vi "RemoteVI Origin Message.vi"(0 "origin":cluster{"x":i32, "y":i32}) -> (4 "frame":string)   [LabVIEW 2020, in "RemoteVI.lvlib"]
doc: "The text message origin x y (docs\\protocol.md 3.3) as a WebSocket text frame (RemoteVI WS Encode Server Frame.vi): where the panel area starts inside the frame - below the menu bar and the toolbar. Every client gets it with the greeting, and all clients again whenever it changes (RemoteVI Send Origin.vi). Pure."
uses:
  RemoteVI.lvlib
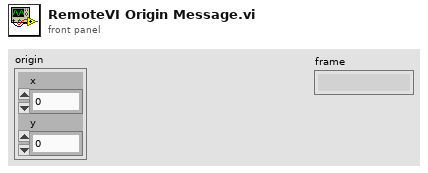
[diagram p1: front panel]
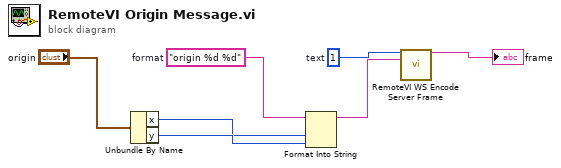
[diagram p0: block diagram]
diagram:
  w6 = u8 1  # text
  w4 = "origin %d %d"  # format
  n1 = Unbundle By Name("origin") -> ("x"=w2:i32, "y"=w3:i32)
  n2 = Format Into String(format string=w4, w2, w3) -> (resulting string=w5:string)  [unwired: 2 in, 1 out]
  n3 = call "RemoteVI WS Encode Server Frame.vi"("opcode"=w6, "payload"=w5) -> ("frame"=→"frame":string)  [unwired: 13 in]
